vi "Host_Event_Loop.vi"(8 "error in (no error)":errorcluster={"status"=FALSE, "code"=0, "source"="\"\""}, 10 "event loop queue":string, 11 "UI references":string) -> (0 "error out":errorcluster={"status"=FALSE, "code"=0, "source"="\"\""}, 2 "status ok":bool, 3 "Host messages":string)   [LabVIEW 2026]
doc: "INTENT: Convert front panel actions into requests. LOGIC: Handle Start/Stop/Manual/ACK button Value Change events; enqueue typed requests only; handle Panel Close."
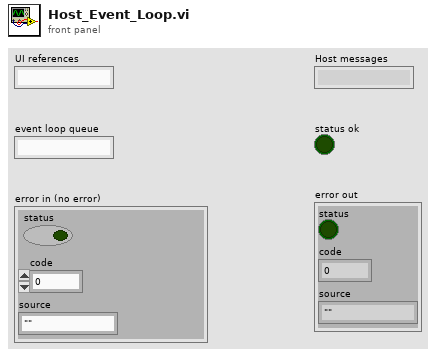
[diagram p1: front panel]
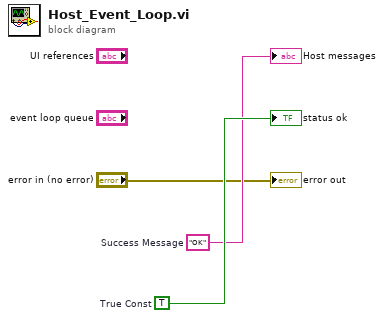
[diagram p0: block diagram]
diagram:
  w3 = TRUE  # True Const
  w2 = "OK"  # Success Message
  "Host messages" <- w2
  "status ok" <- w3
  "error out" <- "error in (no error)"
